vi "VM - Get metrics.vi"(8 "error in":errorcluster, 9 "object":enum32{"variable", "context", "total"}(ring)=enum."total", 10 "name spec":string, 11 "VC Handle":T1=-1) -> (0 "error out":errorcluster, 1 "total size, bytes":u64, 2 "dup name spec":string, 3 "dup VC Handle":T1=-1, 4 "history size, bytes":u64)   [LabVIEW 2021]
doc: "::: CalcExpress Toolkit :::\nCopyright (c) 2000-2026 Konstantin Shifershteyn. All rights reserved."
uses:
  cetypes.llb/VarMan Variable Context Handle.ctl
  cetypes.llb/VarMan Error Code.ctl
  cersrc/celveng32.dll
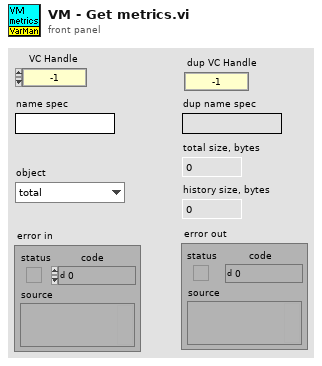
[diagram p1: front panel]
types:
  T1 = typedef "VarMan Variable Context Handle.ctl" = i32
  T2 = typedef "VarMan Error Code.ctl" = u16
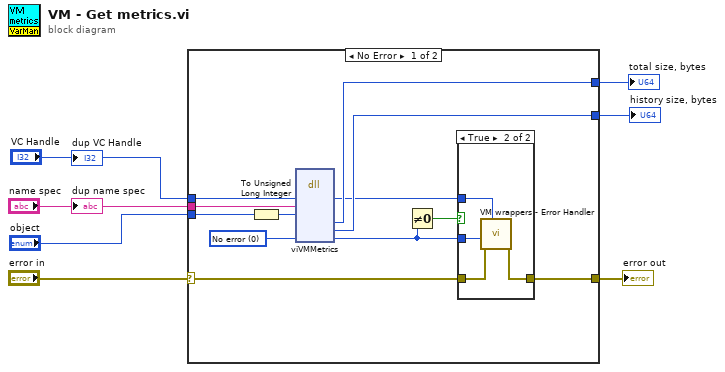
[diagram p0: block diagram]
diagram:
  n1 = case shown="No Error" "error in" {
    selector: "error in" -> [w8 w25]
    tunnel: "object" -> [w19 _]
    tunnel: "name spec" -> [w17 _]
    tunnel: [w16 w25] -> w5
    tunnel: [w15 _] -> w4
    tunnel: [w14 _] -> w3
    tunnel: "VC Handle" -> [w13 _]
    frame No Error {
      w18 = T2 0 items=["No error", "Invalid variable type", "Variable not found", "Variable already exists", "Invalid context handle", "Input error", "Invalid data format", "No history attached", "History already attached", "Invalid history parameters", "Wrong variable name", "Wrong alias name", "Non-unique alias", "Alias not found", "No alias associated", "Alias already associated", "Wrong context name", "Non-unique context name", "Context name not found", "Invalid parameter", "Generic error", "Memory Full", "Unrecognized LV error", "Unknown error code"] ("VarMan error")
      n2 = To Unsigned Long Integer(number=w19) -> (unsigned 32bit integer=w12:u32)
      n3 = dll-call lib="C:/LV Projects/CalcExpress 40 LV2021/vi.lib/addons/CalcExpress/cersrc/celveng*.dll" fn="viVMMetrics"("vch"=w13, "varName"=w17, "object"=w12, "errc"=w18) -> ("vch"=w11:i32, "totalSize"=w15:u64, "histSize"=w14:u64, "errc"=w9:T2)  [unwired: 8 in, 2 out]
      n4 = Not Equal To 0?(x=w9) -> (x != 0?=w10:bool)
      n5 = case shown="True" w10 {
        tunnel: [w20 w24] -> w16
        tunnel: w8 -> [w20 w23]
        tunnel: w9 -> [_ w22]
        tunnel: w11 -> [_ w21]
        frame False {
        }
        frame True {
          n6 = call "VM wrappers - Error Handler.vi"("VC Handle"=w21, "error before"=w23, "VarMan error"=w22) -> ("error out"=w24:errorcluster)  [unwired: 7 in, 1 out]
        }
      }
    }
    frame Error {
    }
  }
  "error out" <- w5
  "total size, bytes" <- w4
  "history size, bytes" <- w3
  "dup VC Handle" <- "VC Handle"
  "dup name spec" <- "name spec"
